vi "libssh2_session_banner_set.vi"(8 "error in (no error)":errorcluster, 10 "banner":string, 11 "session":T1) -> (0 "error out":errorcluster)   [LabVIEW 2017, in "libssh2.lvlib"]
doc: "Set the banner that will be sent to the server when a session is established."
uses:
  libssh2.lvlib
  Session Refnum.ctl
  Not A Session.vi
  <vilib>/Utility/error.llb/Error Cluster From Error Code.vi
  Global Settings.vi
  Read Session Refnum.vi
  <vilib>/Utility/semaphor.llb/Acquire Semaphore.vi
  <vilib>/Utility/semaphor.llb/Release Semaphore.vi
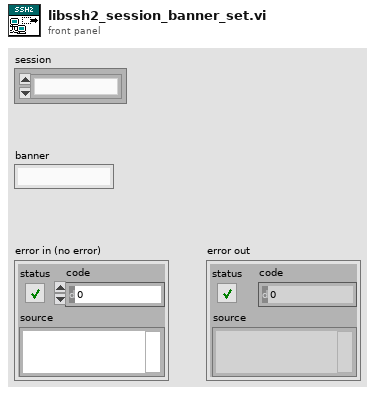
[diagram p1: front panel]
types:
  T1 = typedef "libssh2.lvlib/Session Refnum.ctl" = refnum<k1>
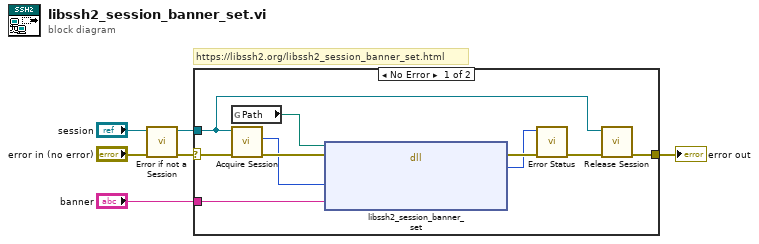
[diagram p0: block diagram]
diagram:
  # "https://libssh2.org/libssh2_session_banner_set.html"
  n1 = call "Error if not a Session.vi"("error in (no error)"="error in (no error)", "session"="session") -> ("error out"=w4:errorcluster, "session out"=w2:T1)  [unwired: 8 in]
  n2 = case shown="No Error" w4 {
    selector: w4 -> [w7 w17]
    tunnel: [w9 w17] -> w6
    tunnel: w2 -> [w8 _]
    tunnel: "banner" -> [w12 _]
    frame No Error {
      n3 = global read "Global Settings.vi" "Path"() -> (w13:path)
      n4 = call "Acquire Session.vi"("error in (no error)"=w7, "session"=w8) -> ("error out"=w15:errorcluster, "LIBSSH2_SESSION*"=w14:u64)  [unwired: 7 in, 1 out]
      n5 = dll-call lib="?" fn="libssh2_session_banner_set"(path in=w13, error in=w15, "session"=w14, "banner"=w12) -> (error out=w16:errorcluster, "return value"=w10:i32)  [unwired: 3 in, 1 out]
      n6 = call "Error Status.vi"("error in (no error)"=w16, "return value"=w10) -> ("error out"=w11:errorcluster)  [unwired: 8 in, 1 out]
      n7 = call "Release Session.vi"("error in (no error)"=w11, "session"=w8) -> ("error out"=w9:errorcluster)  [unwired: 9 in]
    }
    frame Error {
    }
  }
  "error out" <- w6
